vi "Neopixel_Control_Ex.vi"() -> ()   [LabVIEW 2026]
panel:
  out "error out":errorcluster
  in  "Stop Button":bool
  out "respuesta":string
  in  "Color Box":u32(colorbox)
  in  "VISA resource name":refnum<visa-resource-name>
  in  "Opcion":u8
  # "Ejemplo: Neopixel Control"
  # "Descripción: enciende todos los Pixeles del mismo color"
  # "Configuracion"
  # "Indicadores"
  # "Control"
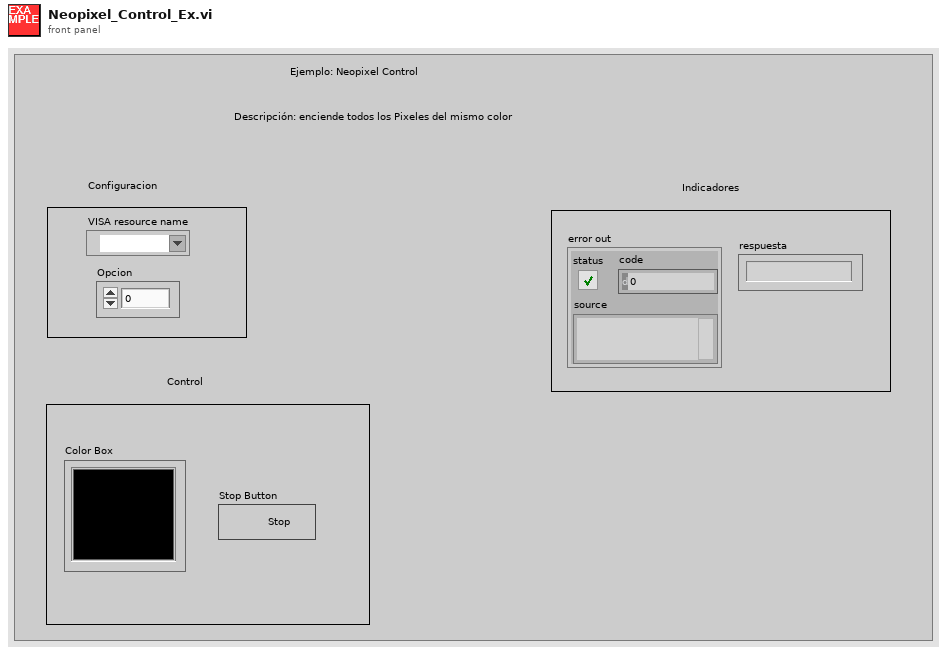
[diagram p1: front panel]
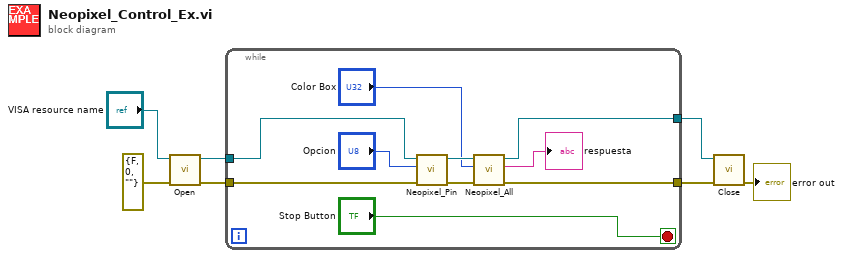
[diagram p0: block diagram]
diagram:
  n1 = call "Open.vi"("error in (no error)"=errorcluster {"status"=FALSE, "code"=0, "source"=""}, "VISA resource name"="VISA resource name") -> ("error out"=w6:errorcluster, "VISA resource name out"=w7:refnum<visa-resource-name>)  [unwired: 8 in]
  n2 = while {
    tunnel: w7 -> [w17]
    tunnel: [w13] -> w3
    tunnel: w6 -> [w16]
    tunnel: [w12] -> w2
    stop <- "Stop Button" stop-if-true
    n3 = call "Neopixel_Pin.vi"("error in (no error)"=w16, "Opcion"="Opcion", "VISA resource name"=w17) -> ("error out"=w10:errorcluster, "VISA resource name out"=w14:refnum<visa-resource-name>)  [unwired: 6 in, 1 out]
    n4 = call "Neopixel_All.vi"("error in (no error)"=w10, "Color Box"="Color Box", "VISA resource name"=w14) -> ("error out"=w12:errorcluster, "respuesta"=→"respuesta":string, "VISA resource name out"=w13:refnum<visa-resource-name>)  [unwired: 6 in]
  }
  n5 = call "Close.vi"("error in (no error)"=w2, "VISA resource name"=w3) -> ("error out"=→"error out":errorcluster)  [unwired: 9 in]
